vi "DiffDriveTrainSim_GetDynamics.vi"(9 "U":T1, 10 "X":T1, 11 "Info":variant) -> (0 "Error":bool, 3 "XDOT":T1)   [LabVIEW 2019, in "Trajectory_Library.lvlib"]
doc: "Diff Drive Train Sim internal call back function to get dynamics. This is used by the Update function.\n\nInputs:\n - Info -- Extra data variant value containing:\n Matrix A\n Matrix B\n Double CurrentGear\n Double OriginalGear\n Double m_rb \n - X -- X matrix\n - U -- U matrix\n\nOutputs:\n - xDot\n - Error -- If TRUE, an error occured."
uses:
  Trajectory_Library.lvlib
  <vilib>/Analysis/Matrix/NI_Matrix.lvlib
  <vilib>/Analysis/Matrix/Numeric/Multiply/Multiply - RM,R.vi
  <vilib>/Analysis/Matrix/Datatypes/RealMatrix.ctl
  <vilib>/Analysis/NI_AALBase.lvlib
  <vilib>/Analysis/baseanly.llb/Real A x B.vi
  <vilib>/Analysis/Matrix/Numeric/Add/Add - RM,RM.vi
  Enum/DIFF_DRIVE_TRAIN_SIM_STATE_ENUM.ctl
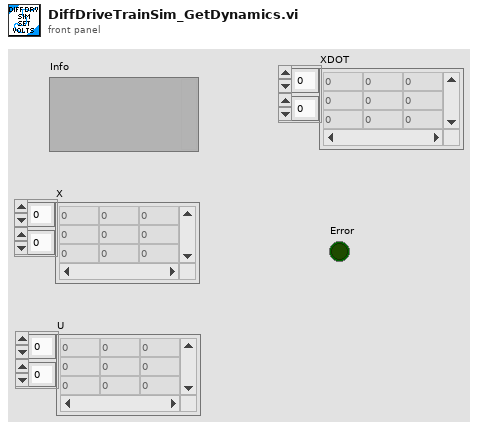
[diagram p1: front panel]
types:
  T1 = typedef "NI_Matrix.lvlib/RealMatrix.ctl" = dbl[][]
  T2 = typedef "Trajectory_Library.lvlib/DIFF_DRIVE_TRAIN_SIM_STATE_ENUM.ctl" = enum16{"X_POS", "Y_POS", "HEADING", "LEFT_VEL", "RIGHT_VEL", "LEFT_DIST", "RIGHT_DIST"}
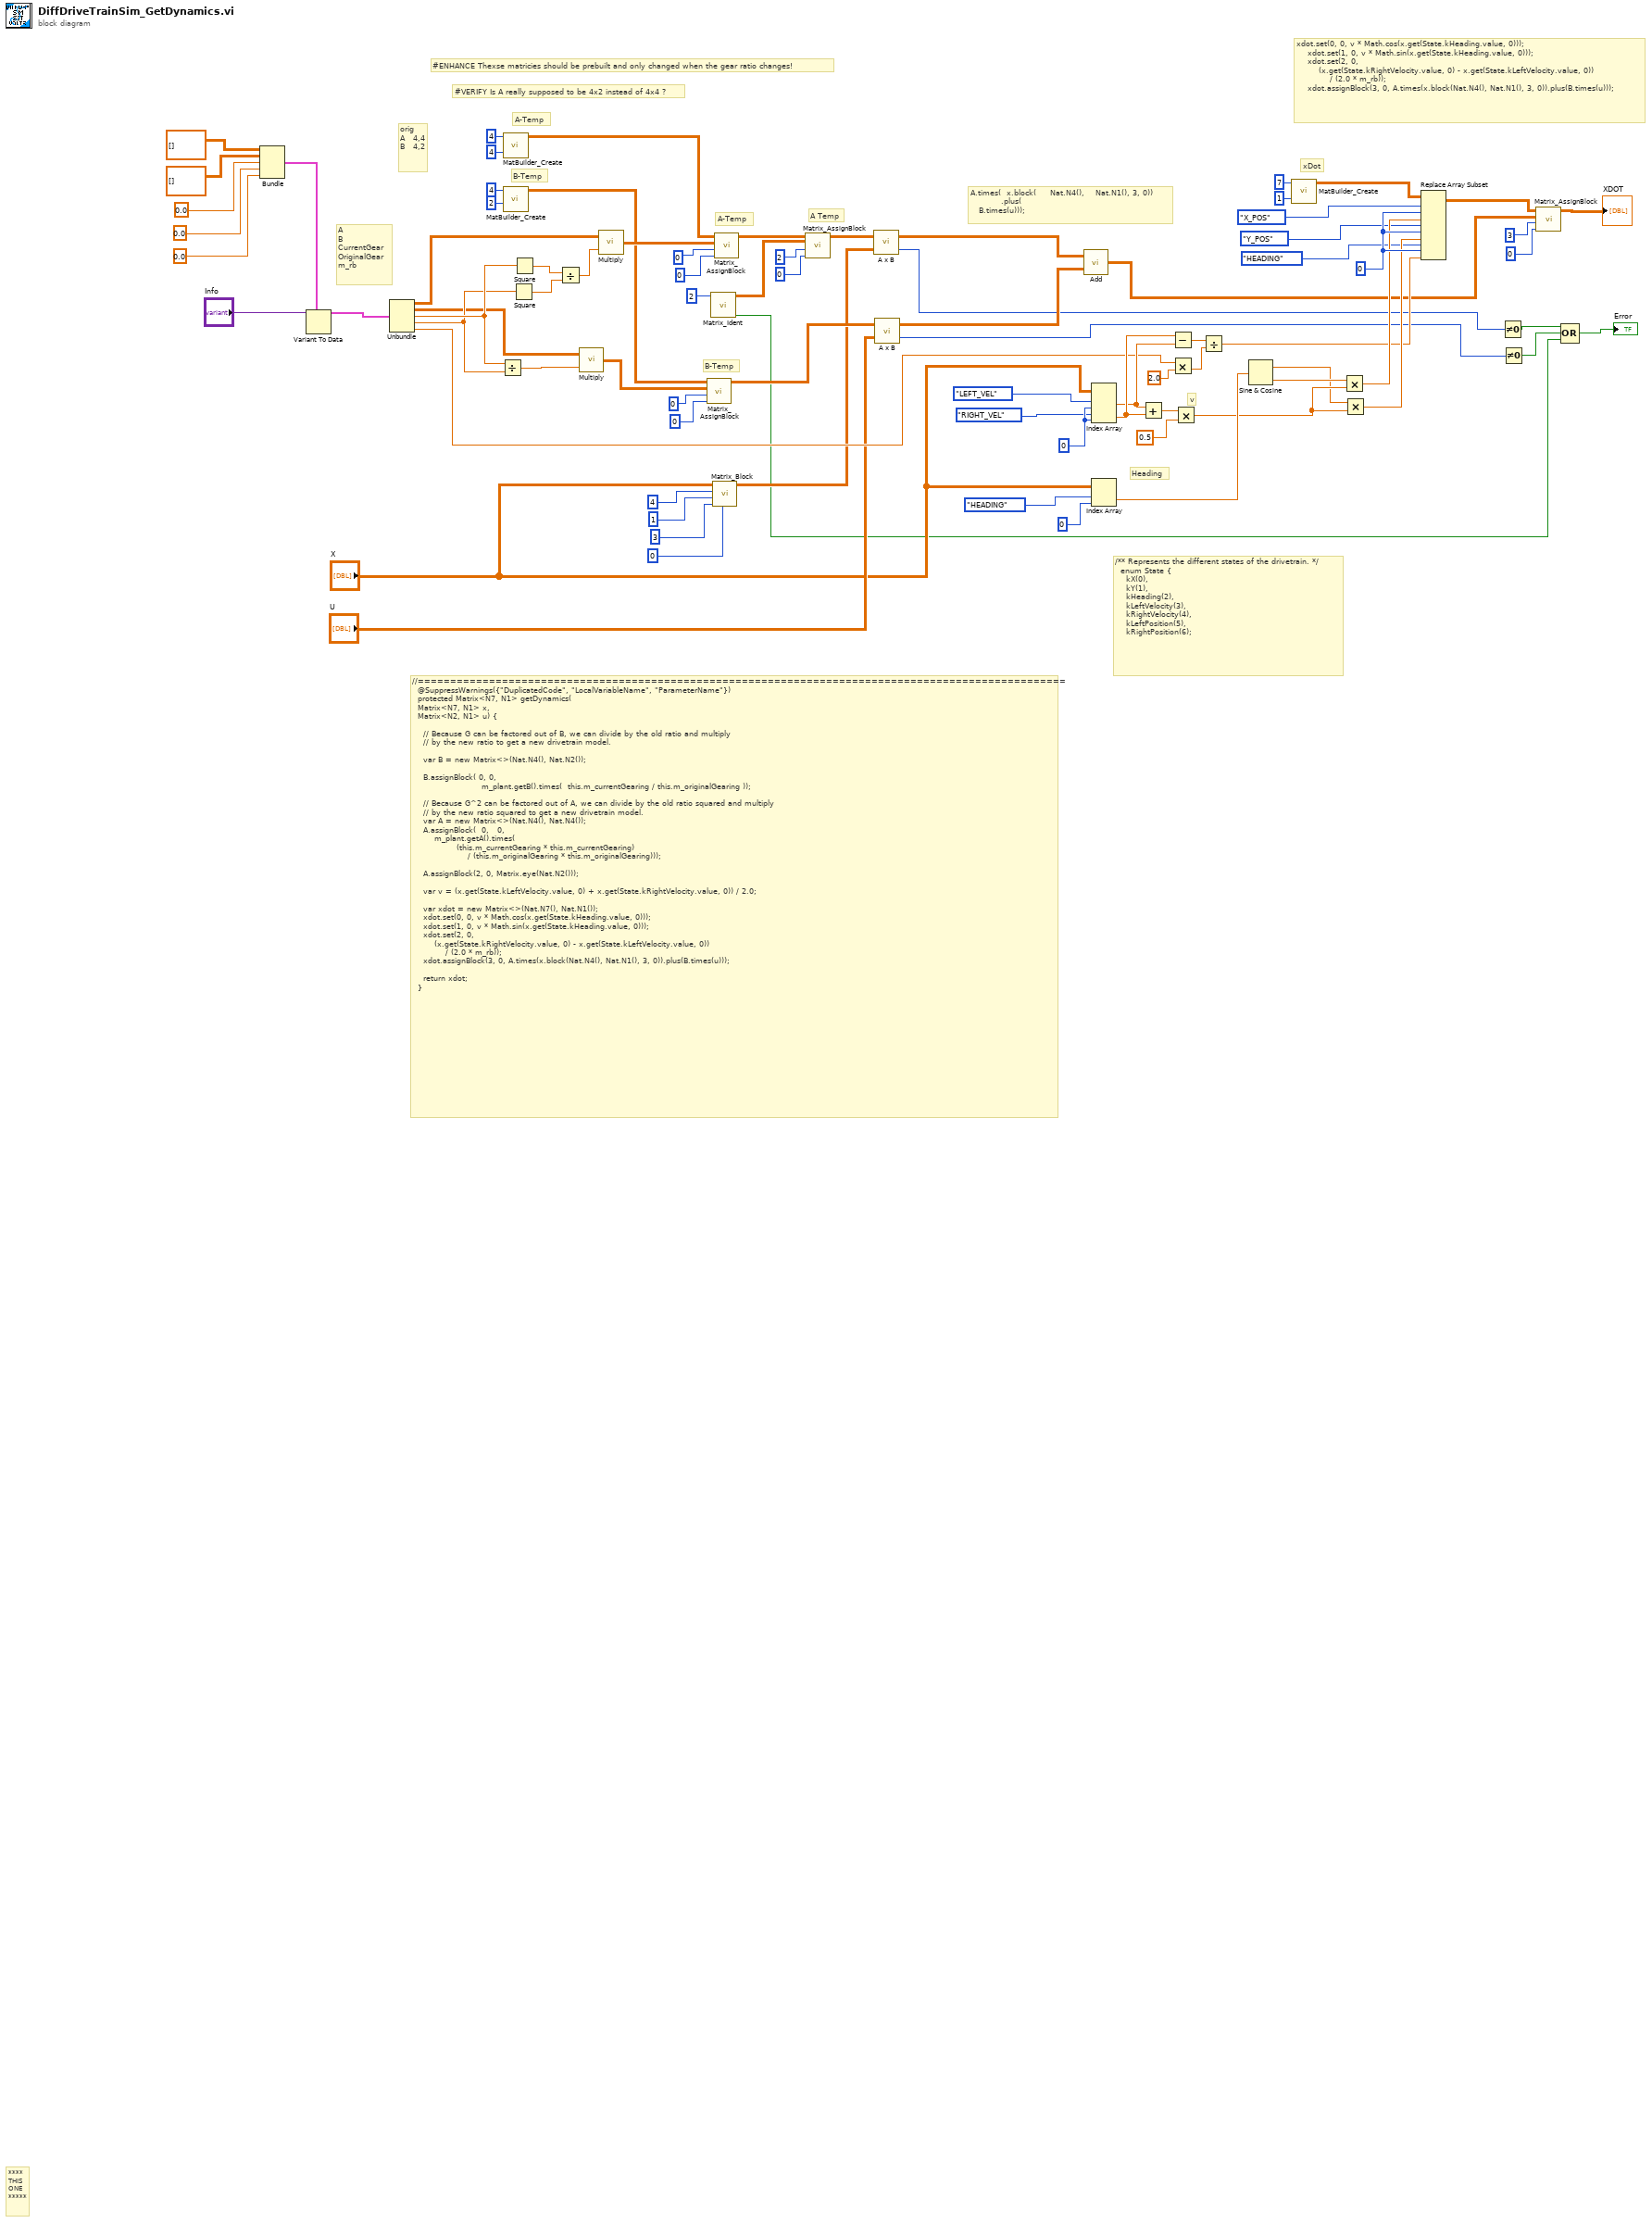
[diagram p0: block diagram]
diagram:
  w56 = 0 ("index (col)")
  w61 = 0 ("index (col)")
  # "orig \nA   4,4\nB   4,2"
  # "B-Temp"
  # "A-Temp"
  # "A.times(  x.block(     Nat.N4(),    Nat.N1(), 3, 0))\n           .plus(  \n   B.times(u)));"
  # "Heading"
  # "v"
  # "xdot.set(0, 0, v * Math.cos(x.get(State.kHeading.value, 0)));\n    xdot.set(1, 0, v * Math.sin(x.get(State.kHeading.value, 0)));\n    xdot.set(2, 0,\n        (x.get(State.kRightVelocity.value, 0) - x.get(State.kLeftVelocity.value, 0))\n            / (2.0 * m_rb));\n    xdot.assignBlock(3, 0, A.times(x.block(Nat.N4(), Nat.N1(), 3, 0)).plus(B.times(u)));"
  # "/** Represents the different states of the drivetrain. */\n  enum State {\n    kX(0),\n    kY(1),\n    kHeading(2),\n    kLeftVelocity(3),\n    kRightVelocity(4),\n    kLeftPosition(5),\n    kRightPosition(6);"
  # "xDot"
  # "#VERIFY Is A really supposed to be 4x2 instead of 4x4 ?"
  # "A Temp"
  # "B-Temp"
  # "A-Temp"
  # "A\nB\nCurrentGear\nOriginalGear\nm_rb"
  # "#ENHANCE Thexse matricies should be prebuilt and only changed when the gear ratio changes!"
  # "//====================================================================================================\n  @SuppressWarnings({\"DuplicatedCode\", \"LocalVariableName\", \"ParameterName\"})\n  protected Matrix<N7, N1> getDynamics(\n\t\tMatrix<N7, N1> x, \n\t\tMatrix<N2, N1> u) {\n\n    // Because G can be factored out of B, we can divide by the old ratio and multiply\n    // by the new ratio to get a new drivetrain model.\n\n    var B = new Matrix<>(Nat.N4(), Nat.N2());\n\n    B.assignBlock( 0, 0, \n\t\t                       m_plant.getB().times(  this.m_currentGearing / this.m_originalGearing ));\n\n    // Because G^2 can be factored out of A, we can divide by the old ratio squared and multiply\n    // by the new ratio squared to get a new drivetrain model.\n    var A = new Matrix<>(Nat.N4(), Nat.N4());\n    A.assignBlock(  0,   0,\n        m_plant.getA().times(\n                (this.m_currentGearing * this.m_currentGearing)\n                    / (this.m_originalGearing * this.m_originalGearing)));\n\n    A.assignBlock(2, 0, Matrix.eye(Nat.N2()));\n\n    var v = (x.get(State.kLeftVelocity.value, 0) + x.get(State.kRightVelocity.value, 0)) / 2.0;\n\n    var xdot = new Matrix<>(Nat.N7(), Nat.N1());\n    xdot.set(0, 0, v * Math.cos(x.get(State.kHeading.value, 0)));\n    xdot.set(1, 0, v * Math.sin(x.get(State.kHeading.value, 0)));\n    xdot.set(2, 0,\n        (x.get(State.kRightVelocity.value, 0) - x.get(State.kLeftVelocity.value, 0))\n            / (2.0 * m_rb));\n    xdot.assignBlock(3, 0, A.times(x.block(Nat.N4(), Nat.N1(), 3, 0)).plus(B.times(u)));\n\n    return xdot;\n  }"
  # "****\nTHIS\nONE\n*****"
  n1 = Bundle("matrix"=T1 [], "matrix"=T1 [], 0.0, 0.0, 0.0) -> (w69:cluster{"matrix":T1, "matrix":T1, dbl, dbl, dbl})  [unwired: 1 in]
  n2 = Variant To Data(type=w69, Variant="Info") -> (data=w68:cluster{"matrix":T1, "matrix":T1, dbl, dbl, dbl})  [unwired: 1 in, 1 out]
  n3 = Unbundle(w68) -> ("matrix"=w78:T1, "matrix"=w76:T1, w82:dbl, w81:dbl, w45:dbl)
  n4 = Divide(x=w82, y=w81) -> (x/y=w75:dbl)
  n5 = call "MatBuilder_Create.vi"("Columns"=4, "Rows"=4) -> ("output matrix"=w33:T1)  [unwired: 9 in]
  n6 = call "MatBuilder_Create.vi"("Columns"=2, "Rows"=4) -> ("output matrix"=w29:T1)  [unwired: 9 in]
  n7 = Square(x=w81) -> (x^2=w79:dbl)
  n8 = Square(x=w82) -> (x^2=w80:dbl)
  n9 = Divide(x=w80, y=w79) -> (x/y=w77:dbl)
  n10 = call-poly <vilib>:"Multiply.vi"("Real Scalar c"=w75, "Real Matrix A"=w76) -> ("A * c"=w28:T1)
  n11 = call-poly <vilib>:"Multiply.vi"("Real Scalar c"=w77, "Real Matrix A"=w78) -> ("A * c"=w32:T1)
  n12 = call "Matrix_AssignBlock.vi"("StartColumn"=0 ("row N"), "StartRow"=0 ("row 1"), "Other Matrix"=w28, "input matrix"=w29) -> ("output matrix"=w18:T1)  [unwired: 7 in]
  n13 = call "Matrix_Ident.vi"("Size"=2 ("matrix size")) -> ("Error"=w7:bool, "output matrix"=w9:T1)  [unwired: 9 in]
  n14 = call "Matrix_Block.vi"("StartColumn"=0, "StartRow"=3, "Columns"=1, "Rows"=4, "input matrix"="X") -> ("output matrix"=w16:T1)  [unwired: 6 in]
  n15 = call "Matrix_AssignBlock.vi"("StartColumn"=0 ("row N"), "StartRow"=0 ("row 1"), "Other Matrix"=w32, "input matrix"=w33) -> ("output matrix"=w25:T1)  [unwired: 7 in]
  n16 = call "Matrix_AssignBlock.vi"("StartColumn"=0 ("column 1"), "StartRow"=2 ("row 1"), "Other Matrix"=w9, "input matrix"=w25) -> ("output matrix"=w19:T1)  [unwired: 7 in]
  n17 = call-poly <vilib>:"A x B.vi"("B"=w16, "A"=w19) -> ("error"=w39:i32, "A x B"=w40:T1)
  n18 = call-poly <vilib>:"A x B.vi"("B"="U", "A"=w18) -> ("error"=w38:i32, "A x B"=w41:T1)
  n19 = call-poly <vilib>:"Add.vi"("Real Matrix B"=w41, "Real Matrix A"=w40) -> ("A + B"=w11:T1)
  n20 = Index Array(array="X", index (row) #1=DIFF_DRIVE_TRAIN_SIM_STATE_ENUM."LEFT_VEL" ("DIFF_DRIVE_TRAIN_SIM_STATE"), index (col) #1=w61, index (row) #2=DIFF_DRIVE_TRAIN_SIM_STATE_ENUM."RIGHT_VEL" ("DIFF_DRIVE_TRAIN_SIM_STATE"), index (col) #2=w61) -> (element #1=w49:dbl, element #2=w50:dbl)
  n21 = Index Array(array="X", index (row)=DIFF_DRIVE_TRAIN_SIM_STATE_ENUM."HEADING" ("DIFF_DRIVE_TRAIN_SIM_STATE"), index (col)=0) -> (element=w55:dbl)
  n22 = Add ("Add.vi")(x=w49, y=w50) -> (x+y=w60:dbl)
  n23 = Subtract ("Subtract.vi")(x=w50, y=w49) -> (x-y=w44:dbl)
  n24 = Multiply(x=w45, y=2.0) -> (x*y=w47:dbl)
  n25 = Multiply ("Multiply.vi")(x=w60, y=0.5) -> (x*y=w54:dbl)
  n26 = Divide(x=w44, y=w47) -> (x/y=w43:dbl)
  n27 = Sine & Cosine(0:w55) -> (1:w34:dbl, 2:w53:dbl)
  n28 = call "MatBuilder_Create.vi"("Columns"=1, "Rows"=7) -> ("output matrix"=w57:T1)  [unwired: 9 in]
  n29 = Multiply ("Multiply.vi")(x=w53, y=w54) -> (x*y=w52:dbl)
  n30 = Multiply ("Multiply.vi")(x=w34, y=w54) -> (x*y=w51:dbl)
  n31 = Replace Array Subset(array=w57, new element #1=w52, index (row) #1=DIFF_DRIVE_TRAIN_SIM_STATE_ENUM."X_POS" ("DIFF_DRIVE_TRAIN_SIM_STATE"), index (col) #1=w56, new element #2=w51, index (row) #2=DIFF_DRIVE_TRAIN_SIM_STATE_ENUM."Y_POS" ("DIFF_DRIVE_TRAIN_SIM_STATE"), index (col) #2=w56, new element #3=w43, index (row) #3=DIFF_DRIVE_TRAIN_SIM_STATE_ENUM."HEADING" ("DIFF_DRIVE_TRAIN_SIM_STATE"), index (col) #3=w56) -> (w22:T1)
  n32 = Not Equal To 0?(x=w39) -> (x != 0?=w37:bool)
  n33 = Not Equal To 0?(x=w38) -> (x != 0?=w36:bool)
  n34 = call "Matrix_AssignBlock.vi"("StartColumn"=0 ("row N"), "StartRow"=3 ("row N"), "Other Matrix"=w11, "input matrix"=w22) -> ("output matrix"=→"XDOT":T1)  [unwired: 7 in]
  n35 = Compound Arithmetic op=OR(w37, w36, w7) -> (→"Error":bool)
